vi "PathPlanner_PathFinder_ExtractPath.vi"(8 "error in (no error)":errorcluster) -> (0 "error out":errorcluster)   [LabVIEW 2019, in "PathPlanner24.lvlib"]
doc: "Internal function. Not to be used by end users."
uses:
  PathPlanner24.lvlib
  <vilib>/Rock Robotics/WPI/ThirdParty/JAS_Junk/TrajLib/TypeDef/TRANSLATION2D.ctl
  TypeDef/PathPlannerFinderGridPosition.ctl
  PathPlanner_GridPosition_Get.vi
  <vilib>/Rock Robotics/WPI/ThirdParty/JAS_Junk/TrajLib/Translation2d_Create.vi
  <vilib>/Rock Robotics/WPI/ThirdParty/JAS_Junk/TrajLib/Translation2d_Times.vi
  PathPlanner_GridPosition_New.vi
  <vilib>/Rock Robotics/WPI/ThirdParty/JAS_Junk/TrajLib/Util_CalcDist.vi
  <vilib>/Rock Robotics/WPI/ThirdParty/JAS_Junk/TrajLib/Rotation2d_GetAngleCosSin.vi
  <vilib>/Rock Robotics/WPI/ThirdParty/JAS_Junk/TrajLib/Translation2d_GetXY.vi
  <vilib>/Rock Robotics/WPI/ThirdParty/JAS_Junk/TrajLib/Rotation2d_CreateXY.vi
  <vilib>/robotics/Navigation/shared/MapNode/AbstractDstarNode/NI_Robotics_AbstractDstarNode.lvclass
  C:/Program Files/National Instruments/LabVIEW 2019/vi.lib/robotics/Navigation/shared/MapNode/AbstractAstarNode/NI_Robotics_AbstractAstarNode.lvclass
  PathPlanner_PathFinder_Globals.vi
  <vilib>/robotics/Navigation/shared/WorldMap/OccupancyGridWorldMap/Get Cells in Path.vi
  <vilib>/Rock Robotics/WPI/ThirdParty/JAS_Junk/TrajLib/Trajectory_Library.lvlib
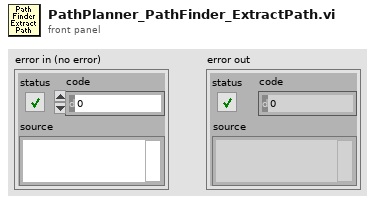
[diagram p1: front panel]
types:
  T1 = typedef "PathPlanner24.lvlib/PathPlannerFinderGridPosition.ctl" = cluster{"X":i32, "Y":i32}
  T2 = typedef "Trajectory_Library.lvlib/TRANSLATION2D.ctl" = cluster{"X":dbl, "Y":dbl}
  T3 = typedef "Trajectory_Library.lvlib/ROTATION2D.ctl" = cluster{"VALUE":dbl, "COS":dbl, "SIN":dbl}
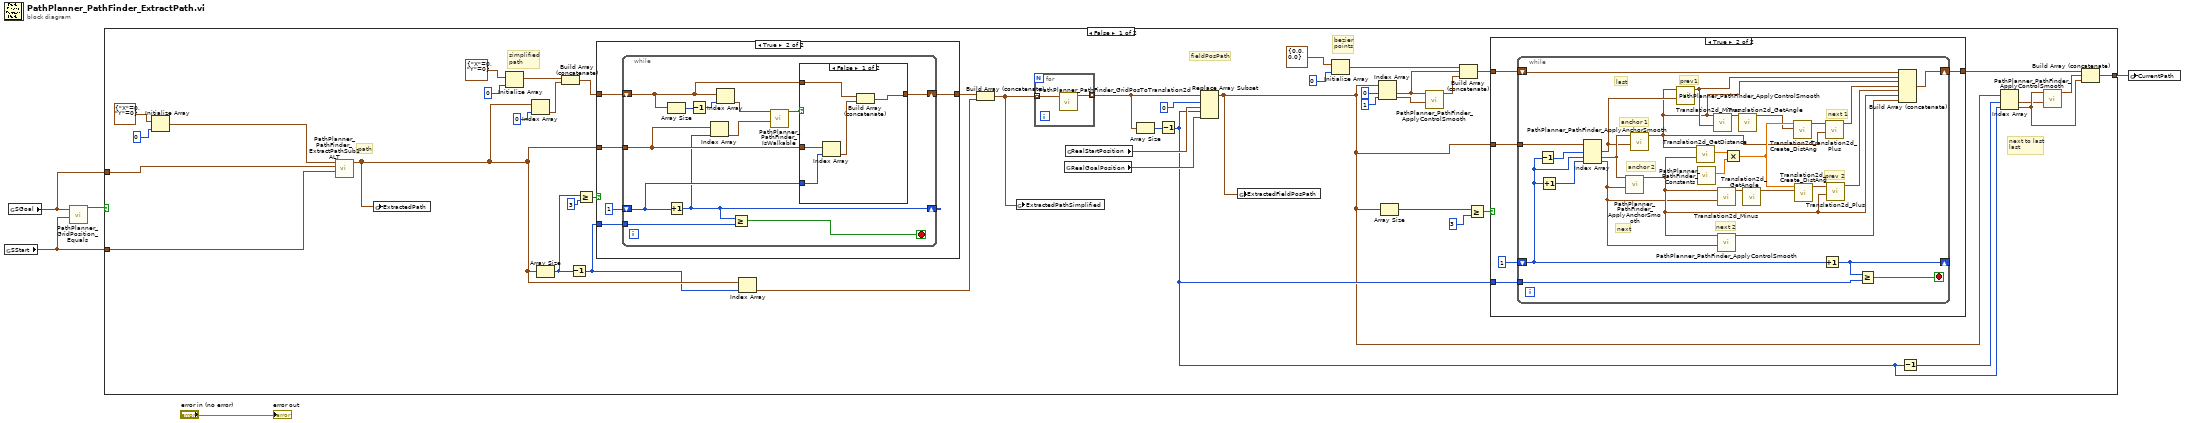
[diagram p0: block diagram]
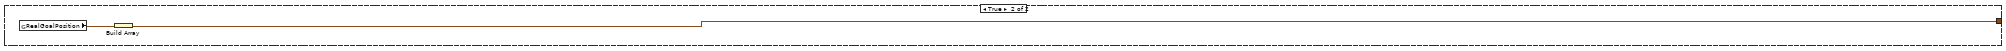
[diagram p5: hidden frame]
diagram:
  n1 = global read "PathPlanner_PathFinder_Globals.vi" "SStart"() -> (w3:T1)
  n2 = global read "PathPlanner_PathFinder_Globals.vi" "SGoal"() -> (w2:T1)
  n3 = call "PathPlanner_GridPosition_Equals.vi"("Other GridPosition"=w3, "GridPosition"=w2) -> ("Equal"=w4:bool)  [unwired: 9 in]
  n4 = case shown="False" w4 {
    tunnel: [w28 w109] -> w1
    tunnel: w3 -> [w24 _]
    tunnel: w2 -> [w25 _]
    frame False {
      # "bezier\npoints"
      # "next to last\nlast"
      # "fieldPosPath"
      # "path"
      # "simplified\npath"
      n5 = Initialize Array(T1 {"X"=0, "Y"=0} ("PathPlannerFinderGridPosition"), 0 ("dimension size")) -> (w26:T1[])
      n6 = call "PathPlanner_PathFinder_ExtractPathSub1ALT.vi"("SStart"=w24, "SGoal"=w25, "PathPoints In"=w26) -> ("Path Points Out"=w20:T1[])  [unwired: 8 in]
      n7 = global write "PathPlanner_PathFinder_Globals.vi" "ExtractedPath"(w20) -> ()
      n8 = Initialize Array(T1 {"X"=0, "Y"=0} ("PathPlannerFinderGridPosition"), 0 ("dimension size")) -> (w23:T1[])
      n9 = Index Array(array=w20, index=0) -> (element=w21:T1)
      n10 = Array Size(array=w20) -> (size(s)=w11:i32)
      n11 = Build Array (concatenate)(w23, w21) -> (w22:T1[])
      n12 = Decrement(x=w11) -> (x-1=w13:i32)
      n13 = Greater Or Equal?(x=w11, y=3) -> (x >= y?=w12:bool)
      n14 = case shown="True" w12 {
        tunnel: [w83 w88] -> w45
        tunnel: w22 -> [w83 w87]
        tunnel: w20 -> [_ w86]
        tunnel: w13 -> [_ w84]
        frame False {
        }
        frame True {
          n15 = while {
            shift-right: [w100] -> w88
            shift-left: w87 -> [w92]
            tunnel: w86 -> [w99]
            shift-right: [w91] -> _
            shift-left: 1 -> [w93]
            tunnel: w84 -> [w89]
            stop <- w90 stop-if-true
            n16 = Array Size(array=w92) -> (size(s)=w97:i32)
            n17 = Increment(x=w93) -> (x+1=w91:i32)
            n18 = Decrement(x=w97) -> (x-1=w96:i32)
            n19 = Index Array(array=w99, index=w91) -> (element=w98:T1)
            n20 = Index Array(array=w92, index=w96) -> (element=w95:T1)
            n21 = Greater Or Equal?(x=w91, y=w89) -> (x >= y?=w90:bool)
            n22 = call "PathPlanner_PathFinder_IsWalkable.vi"("S2"=w98, "S1"=w95) -> ("IsWalkable"=w94:bool)  [unwired: 9 in]
            n23 = case shown="False" w94 {
              tunnel: w92 -> [w105 w106]
              tunnel: [w104 w106] -> w100
              tunnel: w99 -> [w103 _]
              tunnel: w93 -> [w102 _]
              frame False {
                n24 = Index Array(array=w103, index=w102) -> (element=w101:T1)
                n25 = Build Array (concatenate)(w105, w101) -> (w104:T1[])
              }
              frame True {
              }
            }
          }
        }
      }
      n26 = Index Array(array=w20, index=w13) -> (element=w44:T1)
      n27 = Build Array (concatenate)(w45, w44) -> (w27:T1[])
      n28 = global write "PathPlanner_PathFinder_Globals.vi" "ExtractedPathSimplified"(w27) -> ()
      n29 = for {
        tunnel: w27 -> [w108] mode=indexing
        tunnel: [w107] -> w18 mode=indexing
        n30 = call "PathPlanner_PathFinder_GridPosToTranslation2d.vi"("GridPosition"=w108) -> ("RealGridPos"=w107:T2)  [unwired: 10 in]
      }
      n31 = global read "PathPlanner_PathFinder_Globals.vi" "RealGoalPosition"() -> (w40:T2)
      n32 = global read "PathPlanner_PathFinder_Globals.vi" "RealStartPosition"() -> (w42:T2)
      n33 = Array Size(array=w18) -> (size(s)=w41:i32)
      n34 = Decrement(x=w41) -> (x-1=w31:i32)
      n35 = Replace Array Subset(array=w18, new element #1=w42, index #1=0 ("index"), new element #2=w40, index #2=w31) -> (w9:T2[])
      n36 = global write "PathPlanner_PathFinder_Globals.vi" "ExtractedFieldPosPath"(w9) -> ()
      n37 = Initialize Array(T2 {"X"=0.0, "Y"=0.0} ("TRANSLATION2D"), 0 ("dimension size")) -> (w36:T2[])
      n38 = Index Array(array=w9, index #1=0 ("index"), index #2=1 ("index")) -> (element #1=w17:T2, element #2=w16:T2)
      n39 = Array Size(array=w9) -> (size(s)=w7:i32)
      n40 = call "PathPlanner_PathFinder_ApplyControlSmooth.vi"("Other"=w16, "Current"=w17) -> ("Smoothed"=w33:T2)  [unwired: 9 in]
      n41 = Build Array (concatenate)(w36, w17, w33) -> (w34:T2[])
      n42 = Greater Or Equal?(x=w7, y=3) -> (x >= y?=w8:bool)
      n43 = case shown="True" w8 {
        tunnel: w34 -> [w50 w55]
        tunnel: w31 -> [_ w53]
        tunnel: [w50 w52] -> w30
        tunnel: w9 -> [_ w51]
        frame False {
        }
        frame True {
          n44 = while {
            shift-right: [w60] -> w52
            shift-left: w55 -> [w65]
            shift-right: [w82] -> _
            shift-left: 1 -> [w77]
            tunnel: w53 -> [w81]
            tunnel: w51 -> [w79]
            stop <- w80 stop-if-true
            # "prev 2"
            # "last"
            # "next"
            # "next 1"
            # "next 2"
            # "prev1"
            # "anchor 2"
            # "anchor 1"
            n45 = Decrement(x=w77) -> (x-1=w78:i32)
            n46 = Increment(x=w77) -> (x+1=w76:i32)
            n47 = Index Array(array=w79, index #1=w78, index #2=w77, index #3=w76) -> (element #1=w59:T2, element #2=w75:T2, element #3=w56:T2)
            n48 = call "PathPlanner_PathFinder_ApplyAnchorSmooth.vi"("Other"=w56, "Current"=w75) -> ("Smoothed"=w57:T2)  [unwired: 9 in]
            n49 = call "PathPlanner_PathFinder_ApplyAnchorSmooth.vi"("Other"=w59, "Current"=w75) -> ("Smoothed"=w58:T2)  [unwired: 9 in]
            n50 = call "PathPlanner_PathFinder_ApplyControlSmooth.vi"("Other"=w59, "Current"=w58) -> ("Smoothed"=w64:T2)  [unwired: 9 in]
            n51 = call <vilib>:"Translation2d_GetDistance.vi"("other Translation"=w57, "In Translation"=w58) -> ("Distance"=w74:dbl)  [unwired: 9 in]
            n52 = call "PathPlanner_PathFinder_Constants.vi"() -> ("SMOOTHING_CONTROL_PCT"=w73:dbl)  [unwired: 9 in, 2 out]
            n53 = call <vilib>:"Translation2d_Minus.vi"("other Translation"=w64, "In Translation"=w58) -> ("Out Translation"=w71:T2)  [unwired: 9 in]
            n54 = call <vilib>:"Translation2d_Minus.vi"("other Translation"=w56, "In Translation"=w57) -> ("Out Translation"=w69:T2)  [unwired: 9 in]
            n55 = call "PathPlanner_PathFinder_ApplyControlSmooth.vi"("Other"=w56, "Current"=w57) -> ("Smoothed"=w61:T2)  [unwired: 9 in]
            n56 = Multiply(x=w74, y=w73) -> (x*y=w72:dbl)
            n57 = call <vilib>:"Translation2d_GetAngle.vi"("In Translation"=w71) -> ("Angle_Rotation2d"=w70:T3)  [unwired: 10 in]
            n58 = call <vilib>:"Translation2d_GetAngle.vi"("In Translation"=w69) -> ("Angle_Rotation2d"=w68:T3)  [unwired: 10 in]
            n59 = call <vilib>:"Translation2d_Create_DistAng.vi"("Angle"=w70, "Dist"=w72) -> ("TRANSLATION"=w67:T2)  [unwired: 9 in]
            n60 = call <vilib>:"Translation2d_Create_DistAng.vi"("Angle"=w68, "Dist"=w72) -> ("TRANSLATION"=w66:T2)  [unwired: 9 in]
            n61 = Increment(x=w77) -> (x+1=w82:i32)
            n62 = call <vilib>:"Translation2d_Plus.vi"("other Translation"=w58, "In Translation"=w67) -> ("Out Translation"=w63:T2)  [unwired: 9 in]
            n63 = call <vilib>:"Translation2d_Plus.vi"("other Translation"=w57, "In Translation"=w66) -> ("Out Translation"=w62:T2)  [unwired: 9 in]
            n64 = Greater Or Equal?(x=w82, y=w81) -> (x >= y?=w80:bool)
            n65 = Build Array (concatenate)(w65, w64, w58, w63, w62, w57, w61) -> (w60:T2[])
          }
        }
      }
      n66 = Decrement(x=w31) -> (x-1=w32:i32)
      n67 = Index Array(array=w9, index #1=w32, index #2=w31) -> (element #1=w14:T2, element #2=w15:T2)
      n68 = call "PathPlanner_PathFinder_ApplyControlSmooth.vi"("Other"=w14, "Current"=w15) -> ("Smoothed"=w29:T2)  [unwired: 9 in]
      n69 = Build Array (concatenate)(w30, w29, w15) -> (w28:T2[])
    }
    frame True {
      n70 = global read "PathPlanner_PathFinder_Globals.vi" "RealGoalPosition"() -> (w110:T2)
      n71 = Build Array(w110) -> (w109:T2[])
    }
  }
  n72 = global write "PathPlanner_PathFinder_Globals.vi" "CurrentPath"(w1) -> ()
  "error out" <- "error in (no error)"
